vi "configure_cycle_parameters.vi"(7 "Fs":dbl=20000.0 min=0.0 max=50000.0, 8 "error in":errorcluster, 9 "Pulse width":dbl, 10 "Frequency":dbl, 11 "Amplitude":dbl) -> (0 "error out":errorcluster, 3 "output cycle":waveform(dbl)(graph))   [LabVIEW 2025, in "tSNIP.lvlib"]
uses:
  tSNIP.lvlib
  <vilib>/measure/NI_MABase.lvlib
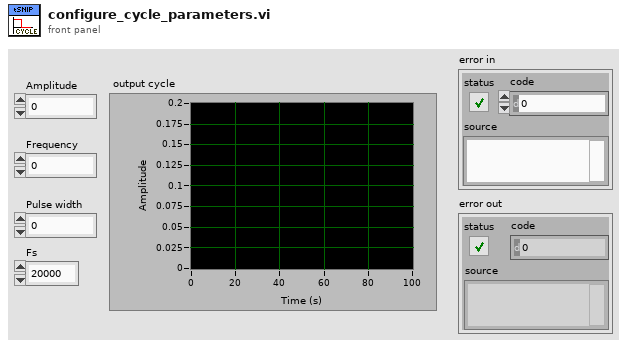
[diagram p1: front panel]
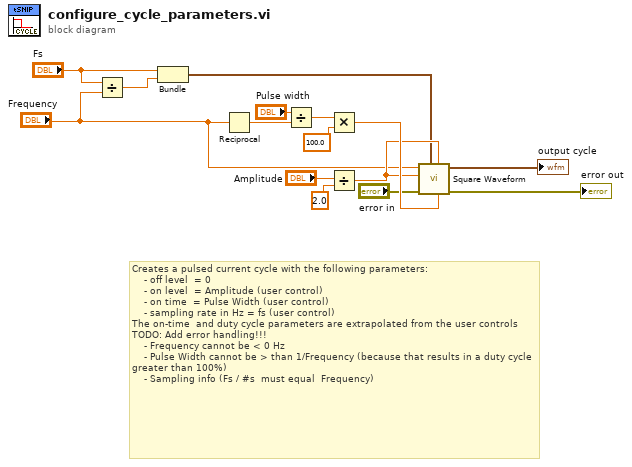
[diagram p0: block diagram]
diagram:
  # "Creates a pulsed current cycle with the following parameters:\n    - off level  = 0\n    - on level  = Amplitude (user control)\n    - on time  = Pulse Width (user control)\n    - sampling rate in Hz = fs (user control)\nThe on-time  and duty cycle parameters are extrapolated from the user controls\nTODO: Add error handling!!!\n    - Frequency cannot be < 0 Hz\n    - Pulse Width cannot be > than 1/Frequency (because that results in a duty cycle greater than 100%)\n    - Sampling info (Fs / #s  must equal  Frequency)"
  n1 = Divide(x="Fs", y="Frequency") -> (x/y=w2:dbl)
  n2 = Bundle("Fs"="Fs", w2) -> (w1:cluster{"Fs":dbl, dbl})  [unwired: 1 in]
  n3 = Reciprocal(x="Frequency") -> (1/x=w14:dbl)
  n4 = Divide(x="Pulse width", y=w14) -> (x/y=w13:dbl)
  n5 = Multiply(x=w13, y=100.0) -> (x*y=w11:dbl)
  n6 = Divide(x="Amplitude", y=2.0) -> (x/y=w6:dbl)
  n7 = call <vilib>:"Square Waveform.vi"("duty cycle (%)"=w11, "offset"=w6, "sampling info"=w1, "error in (no error)"="error in", "amplitude"=w6, "frequency"="Frequency") -> ("error out"=→"error out":errorcluster, "signal out"=→"output cycle":waveform(dbl))  [unwired: 4 in]
